vi "Open Config.vi"(8 "error in (no error)":errorcluster, 11 "Configuration File File In":refnum<class "Configuration File.lvclass">) -> (0 "error out":errorcluster, 3 "Configuration File File Out":refnum<class "Configuration File.lvclass">)   [LabVIEW 2020, in "Configuration File.lvclass"]
doc: "High-level function for opening configuration file data from process class."
uses:
  Configuration File.lvclass
  C:/Git/astemes-triarc-framework/source/Framework/Configuration/Configuration.lvclass
  Base/Base.lvclass/Base.ctl
  Configuration/Protected/Set Config Ref.vi
  Base/Public/Read Config File Path.vi
  Base/Public/Write Config Ref.vi
  Base/Base.lvclass
  <vilib>/Utility/config.llb/NI_LVConfig.lvlib
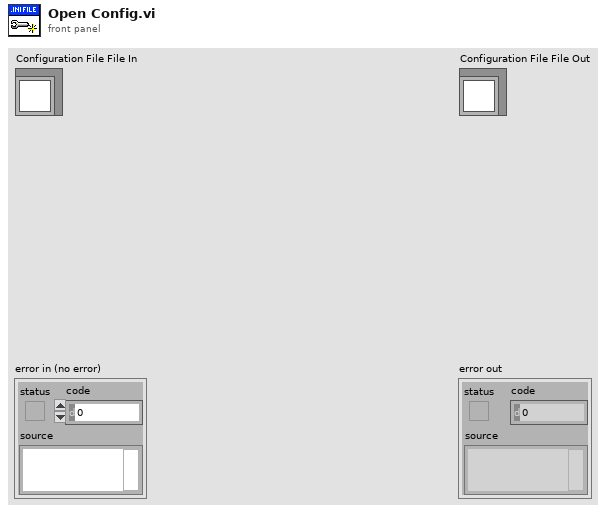
[diagram p1: front panel]
types:
  T1 = typedef "NI_LVConfig.lvlib/Config Data RefNum.ctl" = refnum<k1>
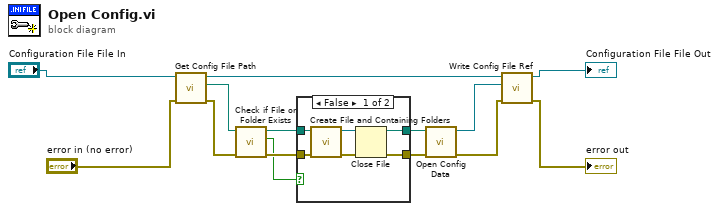
[diagram p0: block diagram]
diagram:
  n1 = call "Get Config File Path.vi"("error in (no error)"="error in (no error)", "Configuration File In"="Configuration File File In") -> ("error out"=w13:errorcluster, "Config File Path"=w6:path, "Configuration File Out"=w14:refnum<class "Configuration File.lvclass">)  [unwired: 7 in]
  n2 = call <vilib>:"Check if File or Folder Exists.vi"("error in (no error)"=w13, "path"=w6) -> ("error out"=w4:errorcluster, "file or folder exists?"=w1:bool, "dup path"=w5:path)  [unwired: 7 in]
  n3 = case shown="False" w1 {
    tunnel: w5 -> [w20 w22]
    tunnel: w4 -> [w19 w21]
    tunnel: [w16 w22] -> w3
    tunnel: [w15 w21] -> w2
    frame False {
      n4 = call <vilib>:"Create File and Containing Folders.vi"("error in (no error)"=w19, "file path"=w20) -> ("error out"=w17:errorcluster, "refnum out"=w18:refnum<file>)  [unwired: 8 in]
      n5 = Close File(refnum=w18, error in=w17) -> (path=w16:path, error out=w15:errorcluster)
    }
    frame True {
    }
  }
  n6 = call <vilib>:"Open Config Data.vi"("error in (no error)"=w2, "configuration file path"=w3) -> ("error out"=w11:errorcluster, "refnum"=w12:T1)  [unwired: 7 in, 1 out]
  n7 = call "Write Config File Ref.vi"("error in (no error)"=w11, "refnum in"=w12, "Configuration File In"=w14) -> ("error out"=→"error out":errorcluster, "Configuration File Out"=→"Configuration File File Out":refnum<class "Configuration File.lvclass">)  [unwired: 7 in]
